vi "NI32LV2612f2ASD5_Untitled 6.vi"() -> ()   [LabVIEW 2026]
panel:
  out "sorted array":dbl[](array[numeric])
  out "Array":dbl[](array[numeric])
  in  "array":dbl[](array[numeric])
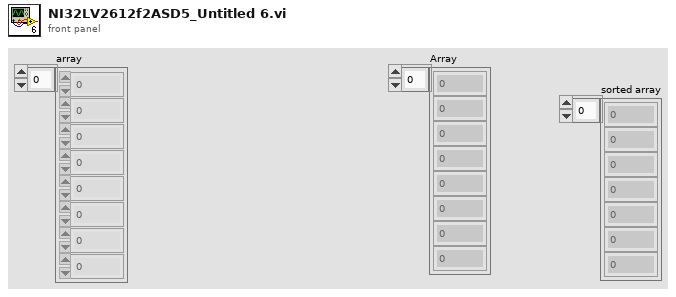
[diagram p1: front panel]
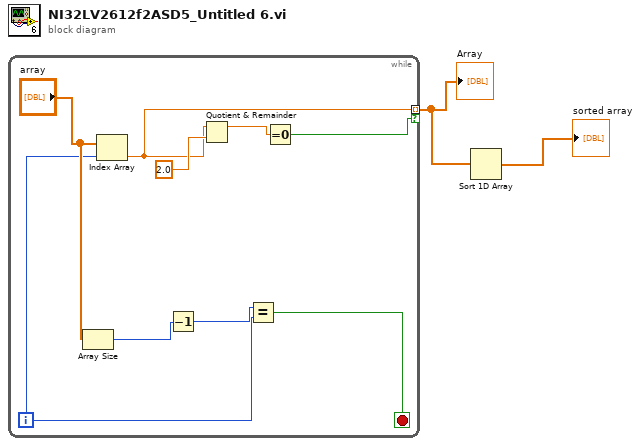
[diagram p0: block diagram]
diagram:
  n1 = while {
    tunnel: [w9] -> w2 mode=indexing if=w8
    i -> [w3]
    stop <- w4 stop-if-true
    n2 = Array Size(array="array") -> (size(s)=w6:i32)
    n3 = Index Array(array="array", index=w3) -> (element=w9:dbl)
    n4 = Decrement(x=w6) -> (x-1=w5:i32)
    n5 = Quotient & Remainder(x=w9, y=2.0) -> (x-y*floor(x/y)=w10:dbl)  [unwired: 1 out]
    n6 = Equal?(x=w5, y=w3) -> (x = y?=w4:bool)
    n7 = Equal To 0?(x=w10) -> (x = 0?=w8:bool)
  }
  "Array" <- w2
  n8 = Sort 1D Array(array=w2) -> (sorted array=→"sorted array":dbl[])
